vi "VIH HelpGen - Reword VI Description for VIs Listing.vi"(11 "String in":string) -> (3 "String out":string)   [LabVIEW 2014]
doc: "::: VI Helpeks :::\nCopyright (c) 2000-2026 Konstantin Shifershteyn. All rights reserved."
panel:
  # "VI Helpeks\nCopyright (c) 2012-2026 Konstantin Shifershteyn"
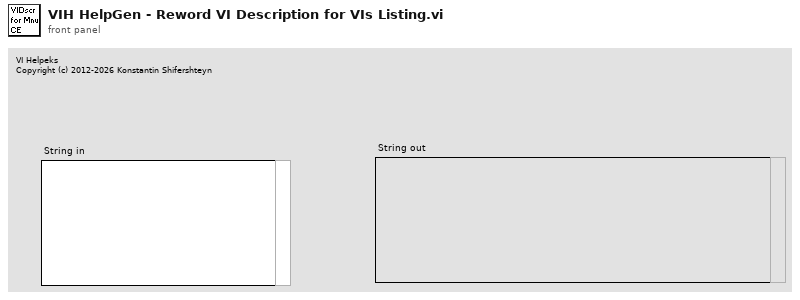
[diagram p1: front panel]
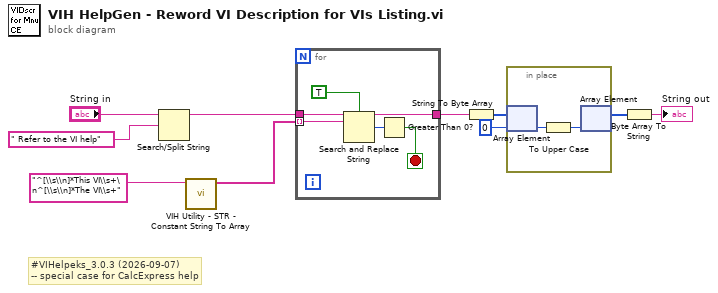
[diagram p0: block diagram]
diagram:
  # "#VIHelpeks_3.0.3 (2026-09-07)\n-- special case for CalcExpress help"
  n1 = Search/Split String(string="String in", search string/char (-)=" Refer to the VI help") -> (substring before match=w8:string)  [unwired: 1 in, 2 out]
  n2 = call "VIH Utility - STR - Constant String To Array.vi"("String in"="^[\\s\\n]*This VI\\s+\n^[\\s\\n]*The VI\\s+") -> ("Array out"=w6:string[])  [unwired: 10 in]
  n3 = for {
    tunnel: w8 -> [w16]
    tunnel: [w14] -> w5
    tunnel: w6 -> [w11] mode=indexing
    stop <- w12 stop-if-true
    n4 = Search and Replace String(case sensitive?=TRUE, input string=w16, search string=w11) -> (result string=w14:string, number of replacements=w13:i32)  [unwired: 5 in, 2 out]
    n5 = Greater Than 0?(x=w13) -> (x > 0?=w12:bool)
  }
  n6 = String To Byte Array(string=w5) -> (unsigned byte array=w4:u8[])
  n7 = in-place {
    n8 = in-place-array #1(w4, 0) -> (w18:u8)
    n9 = To Upper Case(1:w18) -> (0:w17:u8)
    n10 = in-place-array #1(w17) -> (w2:u8[])  [unwired: 1 out]
  }
  n11 = Byte Array To String(unsigned byte array=w2) -> (string=→"String out":string)
